vi "nominal edit api key.vi"(11 "api key in":string) -> (3 "api key out":string)   [LabVIEW 2020, in "nominal core steps.lvlib"]
doc: "Dialog prompt which allows the user to enter their API key.\nNot used as a step.\n\n%docs-exclude%\n<b> </b> <b> </b>"
uses:
  nominal core steps.lvlib
panel:
  in  "reset":bool
  in  "save":bool
  in  "API Key":string
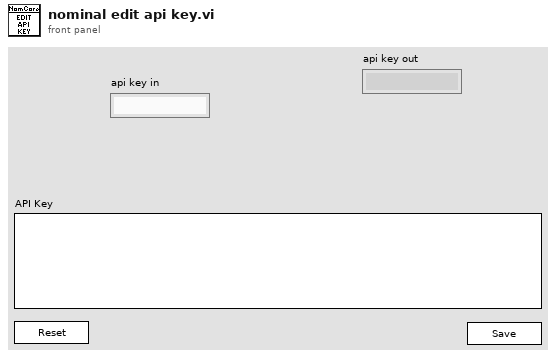
[diagram p1: front panel]
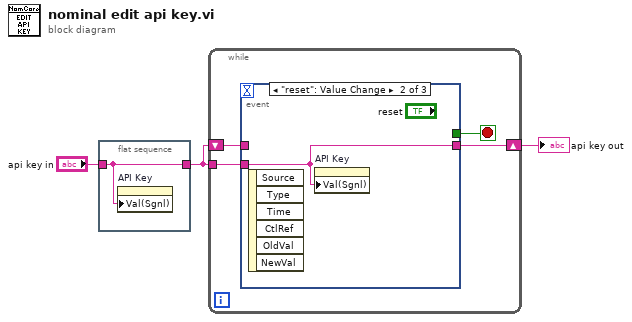
[diagram p0: block diagram]
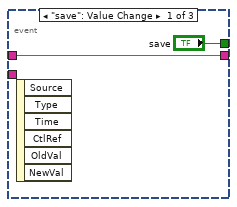
[diagram p2: hidden frame]
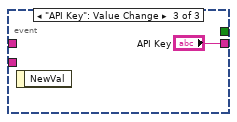
[diagram p3: hidden frame]
diagram:
  n1 = flat-sequence {
    tunnel: [w4] -> w1
    tunnel: "api key in" -> [w4]
    frame #0 {
      n2 = property on="API Key" class="Str"("Val(Sgnl)"=w4) -> ()  [unwired: 2 in, 2 out]
    }
  }
  n3 = while {
    shift-right: [w7] -> w2
    shift-left: w1 -> [w6]
    tunnel: w1 -> [w5]
    stop <- w8 stop-if-true
    n4 = event shown="[1] \"reset\": Value Change" {
      selector: _ -> [_ _ _]
      dyn-events: _ -> [_ _ _]
      timeout: _ -> [_ _ _]
      tunnel: ["save" _ _] -> w8
      tunnel: [w9 w11 "API Key"] -> w7
      tunnel: w6 -> [w9 _ _]
      tunnel: w5 -> [_ w11 _]
      event "save": Value Change {
        n5 = event-data() -> ()  [unwired: 1 in, 6 out]
      }
      event "reset": Value Change {
        n6 = event-data() -> ()  [unwired: 1 in, 6 out]
        n7 = property on="API Key" class="Str"("Val(Sgnl)"=w11) -> ()  [unwired: 2 in, 2 out]
      }
      event "API Key": Value Change {
        n8 = event-data() -> ()  [unwired: 1 in, 1 out]
      }
    }
  }
  "api key out" <- w2
